vi "PathPlanner_ConstraintsZone_FromJSON.vi"(11 "JSON String":string) -> (1 "Exists":bool, 3 "ConstraintZones":T2[](array[typedef]))   [LabVIEW 2019, in "PathPlanner24.lvlib"]
doc: "Create a constraints zone from json\n \nInputs: \n -- JsonString - string - String containing the JSON to parse.\n\nOutputs:\n -- ConstraintsZone - cluster - The constraints zone defined by the given json object\n -- Exists -- boolean -- True if a constraints zone was found and parsed."
uses:
  PathPlanner24.lvlib
  TypeDef/PathPlannerConstraintsZone.ctl
  TypeDef/PathPlannerPathConstraints.ctl
  <vilib>/Rock Robotics/WPI/ThirdParty/JAS_Junk/TrajLib/Trajectory_Library.lvlib
panel:
  in  "constraintZones":T1(array[cluster])
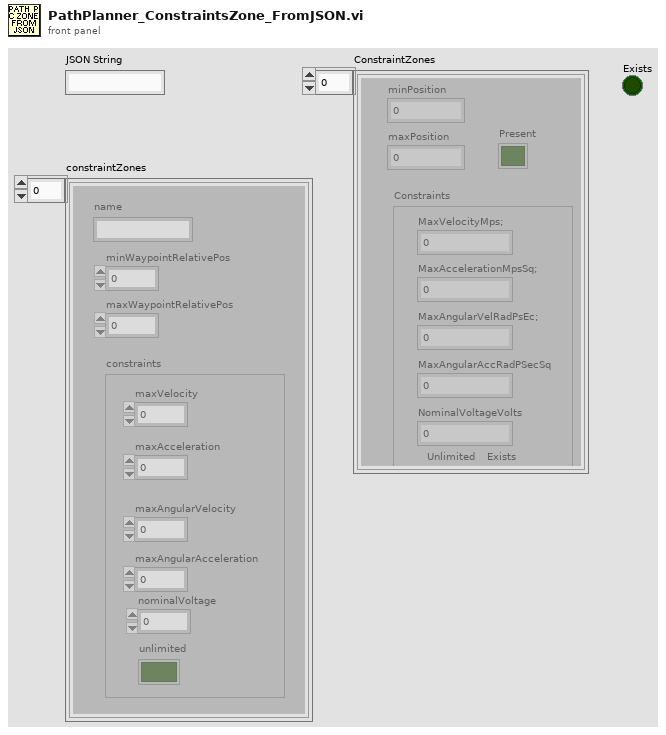
[diagram p1: front panel]
types:
  T1 = cluster{"name":string, "minWaypointRelativePos":dbl, "maxWaypointRelativePos":dbl, "constraints":cluster{"maxVelocity":dbl, "maxAcceleration":dbl, "maxAngularVelocity":dbl, "maxAngularAcceleration":dbl, "nominalVoltage":dbl, "unlimited":bool}}[]
  T2 = typedef "PathPlanner24.lvlib/PathPlannerConstraintsZone.ctl" = cluster{"minPosition":dbl, "maxPosition":dbl, "Constraints":T3, "Present":bool}
  T3 = typedef "PathPlanner24.lvlib/PathPlannerPathConstraints.ctl" = cluster{"MaxVelocityMps;":dbl, "MaxAccelerationMpsSq;":dbl, "MaxAngularVelRadPsEc;":dbl, "MaxAngularAccRadPSecSq":dbl, "Exists":bool, "Unlimited":bool, "NominalVoltageVolts":dbl}
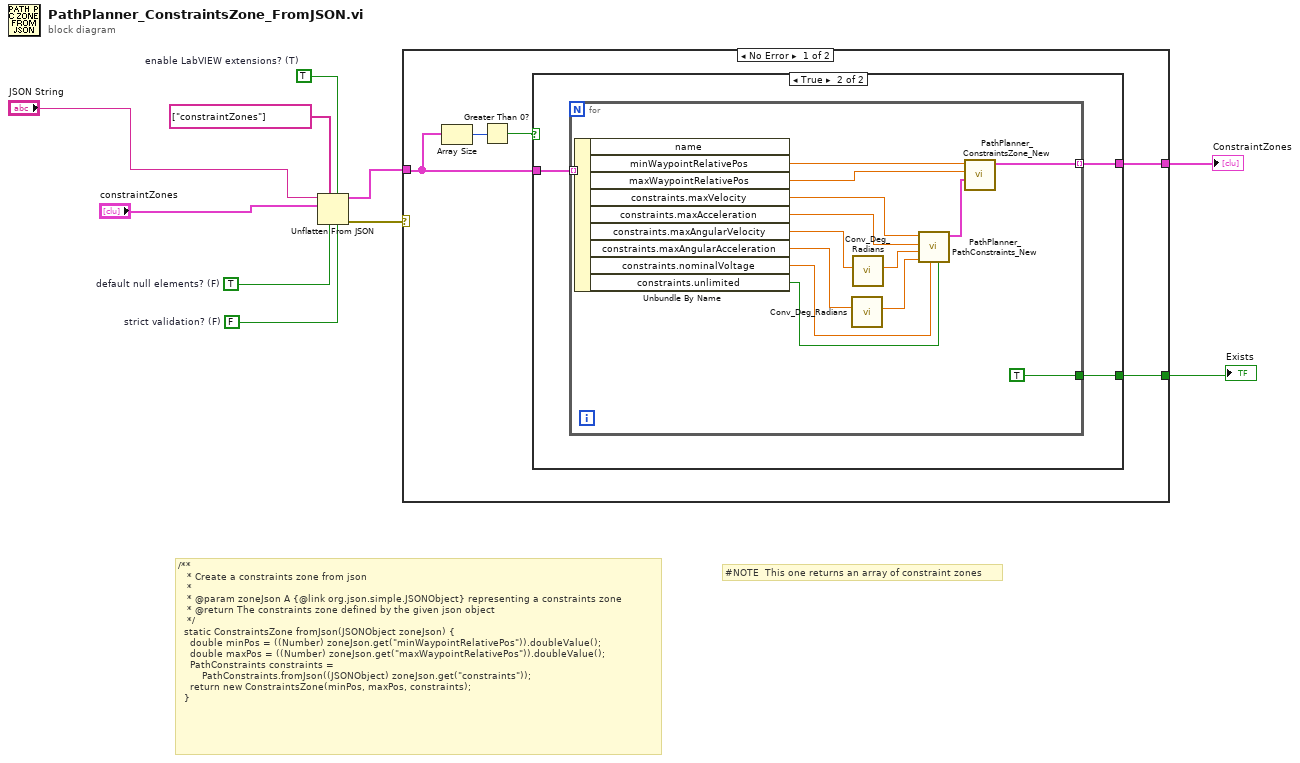
[diagram p0: block diagram]
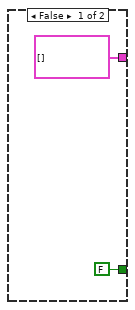
[diagram p2: hidden frame]
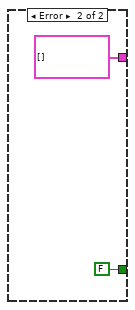
[diagram p3: hidden frame]
diagram:
  w5 = FALSE  # strict validation? (F)
  w6 = TRUE  # default null elements? (F)
  w7 = TRUE  # enable LabVIEW extensions? (T)
  # "#NOTE  This one returns an array of constraint zones"
  # "/**\n   * Create a constraints zone from json\n   *\n   * @param zoneJson A {@link org.json.simple.JSONObject} representing a constraints zone\n   * @return The constraints zone defined by the given json object\n   */\n  static ConstraintsZone fromJson(JSONObject zoneJson) {\n    double minPos = ((Number) zoneJson.get(\"minWaypointRelativePos\")).doubleValue();\n    double maxPos = ((Number) zoneJson.get(\"maxWaypointRelativePos\")).doubleValue();\n    PathConstraints constraints =\n        PathConstraints.fromJson((JSONObject) zoneJson.get(\"constraints\"));\n    return new ConstraintsZone(minPos, maxPos, constraints);\n  }"
  n1 = Unflatten From JSON(path=string[] ["constraintZones"] ("path 5"), enable LabVIEW extensions? (T)=w7, JSON string="JSON String", type and defaults="constraintZones", default null elements? (F)=w6, strict validation? (F)=w5) -> (value=w3:T1, error out=w4:errorcluster)  [unwired: 1 in]
  n2 = case shown="No Error" w4 {
    tunnel: w3 -> [w13 _]
    tunnel: [w12 T2[] []] -> w2
    tunnel: [w11 FALSE] -> w1
    frame No Error {
      n3 = Array Size(array=w13) -> (size(s)=w15:i32)
      n4 = Greater Than 0?(x=w15) -> (x > 0?=w14:bool)
      n5 = case shown="True" w14 {
        tunnel: w13 -> [_ w20]
        tunnel: [T2[] [] w19] -> w12
        tunnel: [FALSE w18] -> w11
        frame False {
        }
        frame True {
          n6 = for {
            tunnel: w20 -> [w34] mode=indexing
            tunnel: [w24] -> w19 mode=indexing
            tunnel: [TRUE] -> w18
            n7 = Unbundle By Name(w34) -> ("minWaypointRelativePos"=w33:dbl, "maxWaypointRelativePos"=w32:dbl, "constraints.maxVelocity"=w31:dbl, "constraints.maxAcceleration"=w30:dbl, "constraints.maxAngularVelocity"=w29:dbl, "constraints.maxAngularAcceleration"=w27:dbl, "constraints.nominalVoltage"=w22:dbl, "constraints.unlimited"=w21:bool)  [unwired: 1 out]
            n8 = call <vilib>:"Conv_Deg_Radians.vi"("Degress"=w27) -> ("Radians"=w26:dbl)  [unwired: 10 in]
            n9 = call <vilib>:"Conv_Deg_Radians.vi"("Degress"=w29) -> ("Radians"=w28:dbl)  [unwired: 10 in]
            n10 = call "PathPlanner_PathConstraints_New.vi"("Unlimited"=w21, "NominalVoltage"=w22, "MaxAngularAccRadPSecSq"=w26, "MaxAngularVelRadPsEc;"=w28, "MaxAccelerationMpsSq;"=w30, "MaxVelocityMps;"=w31) -> ("PathPlannerConstraints"=w25:T3)  [unwired: 5 in]
            n11 = call "PathPlanner_ConstraintsZone_New.vi"("Constraints"=w25, "maxPosition"=w32, "minPosition"=w33) -> ("ConstraintsZone"=w24:T2)  [unwired: 8 in]
          }
        }
      }
    }
    frame Error {
    }
  }
  "ConstraintZones" <- w2
  "Exists" <- w1
